vi "Timer_Check.vi"(8 "error in (no error)":errorcluster={"status"=FALSE, "code"=0, "source"="\"\""}, 10 "monotonic now":string, 11 "TimerTicket":string) -> (0 "error out":errorcluster={"status"=FALSE, "code"=0, "source"="\"\""}, 2 "status ok":bool, 3 "Pending/elapsed/expired":string)   [LabVIEW 2026]
doc: "INTENT: Evaluate timer status. LOGIC: Compare deadlines; return event without sleeping."
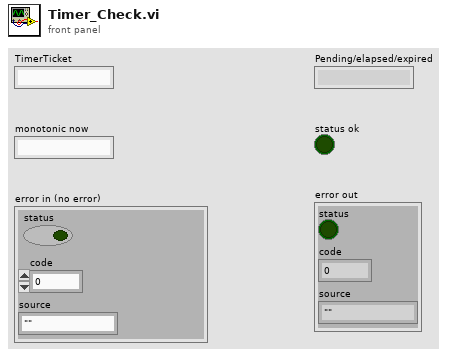
[diagram p1: front panel]
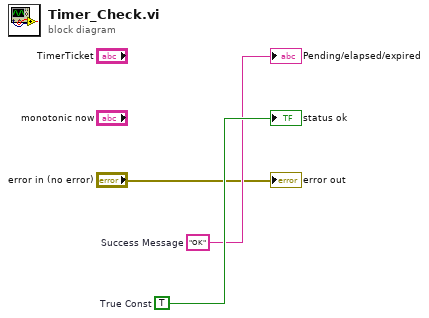
[diagram p0: block diagram]
diagram:
  w3 = TRUE  # True Const
  w2 = "OK"  # Success Message
  "Pending/elapsed/expired" <- w2
  "status ok" <- w3
  "error out" <- "error in (no error)"
